vi "Initialize.vi"(0 "DashboardServer in":refnum<class "Dashboard Server.lvclass">, 5 "error in (no error)":errorcluster) -> (14 "DashboardServer out":refnum<class "Dashboard Server.lvclass">, 19 "error out":errorcluster)   [LabVIEW 2019, in "Dashboard Server.lvclass"]
uses:
  Dashboard Server.lvclass
  Dashboard Server.lvclass/Dashboard Server.ctl
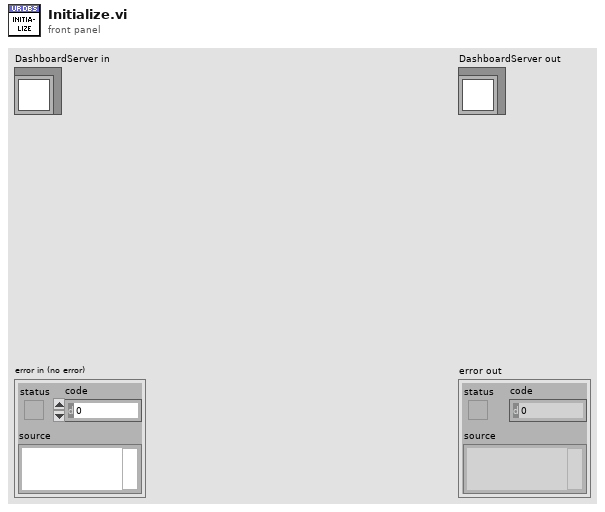
[diagram p1: front panel]
types:
  T1 = typedef "Semaphore RefNum" = refnum<k1>
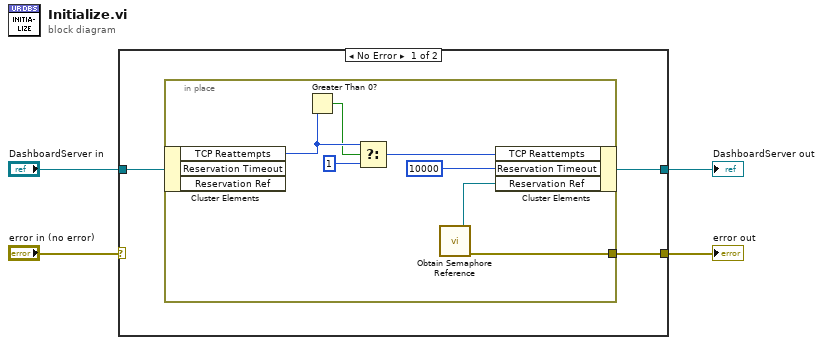
[diagram p0: block diagram]
diagram:
  n1 = case shown="No Error" "error in (no error)" {
    selector: "error in (no error)" -> [_ w16]
    tunnel: [w7 w16] -> w1
    tunnel: [w5 w15] -> w2
    tunnel: "DashboardServer in" -> [w6 w15]
    frame No Error {
      n2 = in-place {
        in-place-border: [w14] -> w7
        n3 = in-place-cluster #1(w6) -> ("TCP Reattempts"=w11:i32)  [unwired: 2 out]
        n4 = Greater Than 0?(x=w11) -> (x > 0?=w9:bool)
        n5 = Select(t=w11, s=w9, f=1) -> (s? t:f=w10:i32)
        n6 = call <vilib>:"Obtain Semaphore Reference.vi"() -> ("error out"=w14:errorcluster, "semaphore"=w13:T1)  [unwired: 5 in, 1 out]
        n7 = in-place-cluster #1("TCP Reattempts"=w10, "Reservation Timeout"=10000 ("reservationTimeout"), "Reservation Ref"=w13) -> (w5:refnum<class "Dashboard Server.lvclass">)
      }
    }
    frame Error {
    }
  }
  "error out" <- w1
  "DashboardServer out" <- w2
